vi "Configure the Function on 1st Display .vi"(5 "Manual Range":dbl format="%#.9e", 7 "Enable Auto Range":bool=TRUE, 8 "error in":errorcluster, 9 "Type for Temperature":u8(ring) items=["J Type", "K Type", "T Type"], 10 "Function":u8(ring) items=["DC Voltage", "AC Voltage", "DC Current", "AC Current", "2-Wire Resistance", "4-Wire Resistance", "Frequency", "Period", "Continuity", "Diode", "Temperature", "Capacitance"], 11 "VISA resource name":refnum<visa-resource-name>) -> (0 "error out":errorcluster, 3 "VISA resource name out":refnum<visa-resource-name>)   [LabVIEW 2012, in "GDM-9052.lvlib"]
uses:
  GDM-9052.lvlib
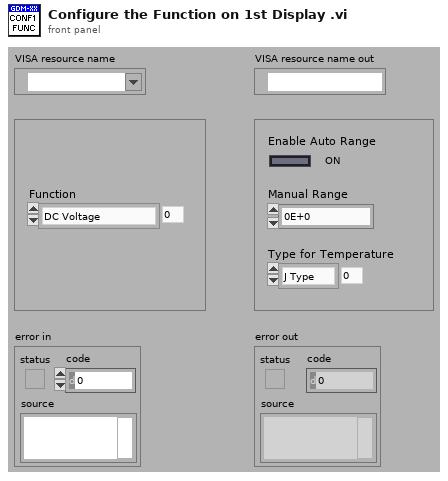
[diagram p1: front panel]
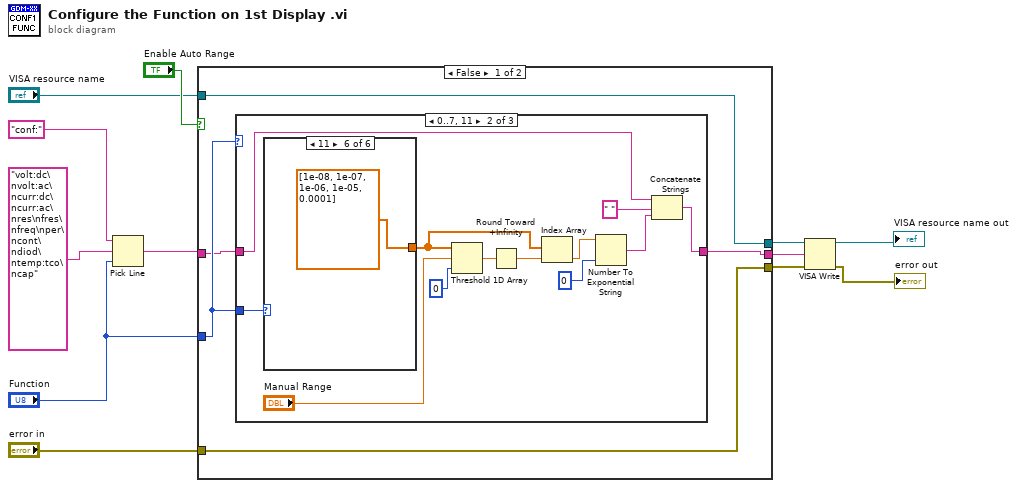
[diagram p0: block diagram]
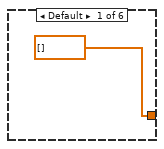
[diagram p3: hidden frame]
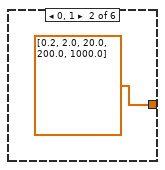
[diagram p4: hidden frame]
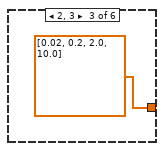
[diagram p5: hidden frame]
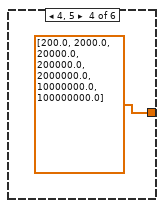
[diagram p6: hidden frame]
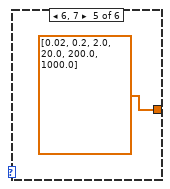
[diagram p7: hidden frame]
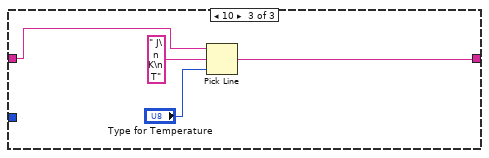
[diagram p8: hidden frame]
diagram:
  n1 = Pick Line(string ("")="conf:", multi-line string="volt:dc\nvolt:ac\ncurr:dc\ncurr:ac\nres\nfres\nfreq\nper\ncont\ndiod\ntemp:tco\ncap", line index="Function") -> (output string=w8:string)
  n2 = case shown="False" "Enable Auto Range" {
    tunnel: "Function" -> [w17 _]
    tunnel: w8 -> [w16 w41]
    tunnel: "VISA resource name" -> [w13 w43]
    tunnel: "error in" -> [w14 w42]
    tunnel: [w13 w43] -> w1
    tunnel: [w14 w42] -> w2
    tunnel: [w15 w41] -> w5
    frame False {
      n3 = case shown="0..7, 11" w17 {
        tunnel: w17 -> [_ w19 _]
        tunnel: w16 -> [w18 w21 w37]
        tunnel: [w18 w20 w38] -> w15
        frame 8, 9, Default {
        }
        frame 0..7, 11 {
          n4 = case shown="11" w19 {
            tunnel: [dbl[] [] dbl[] [0.2, 2.0, 20.0, 200.0, 1000.0] dbl[] [0.02, 0.2, 2.0, 10.0] dbl[] [200.0, 2000.0, 20000.0, 200000.0, 2000000.0, 10000000.0, 100000000.0] dbl[] [0.02, 0.2, 2.0, 20.0, 200.0, 1000.0] dbl[] [1e-08, 1e-07, 1e-06, 1e-05, 0.0001]] -> w26
            frame Default {
            }
            frame 0, 1 {
            }
            frame 2, 3 {
            }
            frame 4, 5 {
            }
            frame 6, 7 {
            }
            frame 11 {
            }
          }
          n5 = Threshold 1D Array(1:0 ("start index (0)"), 2:"Manual Range", 3:w26) -> (0:w28:dbl)
          n6 = Round Toward +Infinity(x=w28) -> (ceil(x): smallest int >= x=w27:dbl)
          n7 = Index Array(array=w26, index=w27) -> (element=w25:dbl)
          n8 = Number To Exponential String(number=w25, precision (6)=i16 0) -> (E-format string=w22:string)  [unwired: 2 in]
          n9 = Concatenate Strings(w21, " " ("string"), w22) -> (w20:string)
        }
        frame 10 {
          n10 = Pick Line(string ("")=w37, multi-line string=" J\n K\n T", line index="Type for Temperature") -> (output string=w38:string)
        }
      }
    }
    frame True {
    }
  }
  n11 = VISA Write(VISA resource name=w1, write buffer=w5, error in (no error)=w2) -> (VISA resource name out=→"VISA resource name out":refnum<visa-resource-name>, error out=→"error out":errorcluster)  [unwired: 1 out]
